vi "~ct - Type of result for 2 numeric args.vi"(6 "error in":bool, 8 "type of right":T1=enum."DBL Number", 9 "type of left":T1=enum."DBL Number") -> (0 "error out":bool, 3 "type of result":T1=enum."DBL Number", 4 "1D-2D sign":i32=-1)   [LabVIEW 2021]
doc: "::: CalcExpress Toolkit :::\nCopyright (c) 2000-2026 Konstantin Shifershteyn. All rights reserved."
uses:
  cetypes.llb/CalcExpress Data Type.ctl
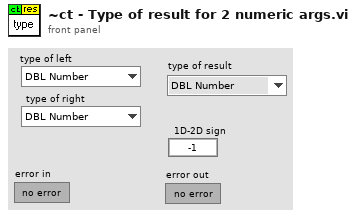
[diagram p1: front panel]
types:
  T1 = typedef "CalcExpress Data Type.ctl" = enum32{"String", "DBL Number", "identifier", "1D Array of DBL", "2D Array of DBL", "CDB Number", "1D Array of CDB", "2D Array of CDB", "1D Array of String", "2D Array of String", "Unknown data type"}
  T2 = enum8{"String", "DBL Number", "identifier", "1D Array of DBL", "2D Array of DBL", "CDB Number", "1D Array of CDB", "2D Array of CDB", "1D Array of String", "2D Array of String", "Unknown data type"}
  T3 = enum32{"String", "DBL Number", "identifier", "1D Array of DBL", "2D Array of DBL", "CDB Number", "1D Array of CDB", "2D Array of CDB", "1D Array of String", "2D Array of String", "Unknown data type"}[][]
  T4 = enum32{"String", "DBL Number", "identifier", "1D Array of DBL", "2D Array of DBL", "CDB Number", "1D Array of CDB", "2D Array of CDB", "1D Array of String", "2D Array of String", "Unknown data type"}
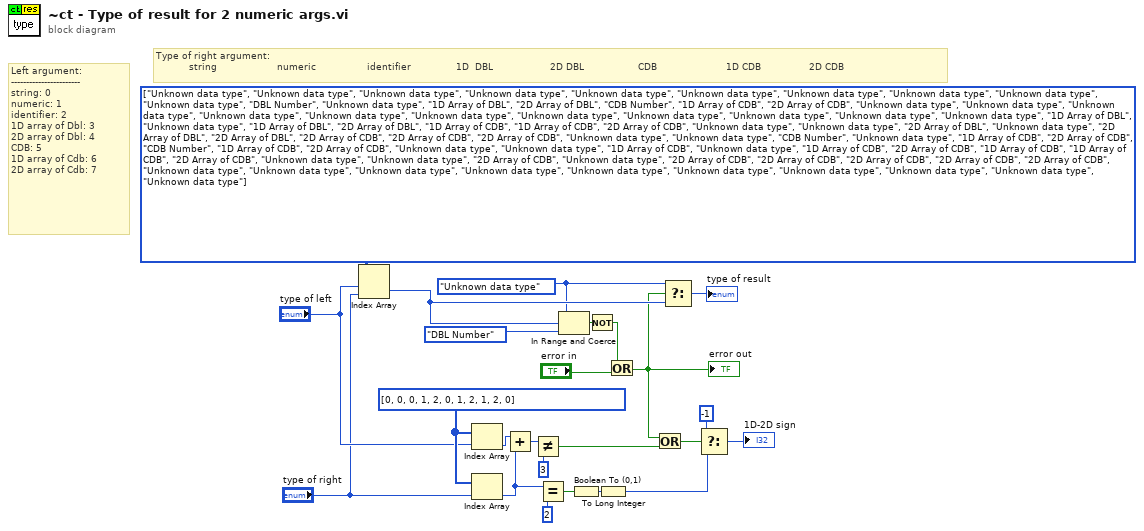
[diagram p0: block diagram]
diagram:
  w7 = i32[] [0, 0, 0, 1, 2, 0, 1, 2, 1, 2, 0]
  w18 = T2."Unknown data type" ("type of result")
  w24 = T3 [[enum."Unknown data type", enum."Unknown data type", enum."Unknown data type", enum."Unknown data type", enum."Unknown data type", enum."Unknown data type", enum."Unknown data type", enum."Unknown data type", enum."Unknown data type"], [enum."Unknown data type", enum."DBL Number", enum."Unknown data type", enum."1D Array of DBL", enum."2D Array of DBL", enum."CDB Number", enum."1D Array of CDB", enum."2D Array of CDB", enum."Unknown data type"], [enum."Unknown data type", enum."Unknown data type", enum."Unknown data type", enum."Unknown data type", enum."Unknown data type", enum."Unknown data type", enum."Unknown data type", enum."Unknown data type", enum."Unknown data type"], [enum."Unknown data type", enum."1D Array of DBL", enum."Unknown data type", enum."1D Array of DBL", enum."2D Array of DBL", enum."1D Array of CDB", enum."1D Array of CDB", enum."2D Array of CDB", enum."Unknown data type"], [enum."Unknown data type", enum."2D Array of DBL", enum."Unknown data type", enum."2D Array of DBL", enum."2D Array of DBL", enum."2D Array of CDB", enum."2D Array of CDB", enum."2D Array of CDB", enum."Unknown data type"], [enum."Unknown data type", enum."CDB Number", enum."Unknown data type", enum."1D Array of CDB", enum."2D Array of CDB", enum."CDB Number", enum."1D Array of CDB", enum."2D Array of CDB", enum."Unknown data type"], [enum."Unknown data type", enum."1D Array of CDB", enum."Unknown data type", enum."1D Array of CDB", enum."2D Array of CDB", enum."1D Array of CDB", enum."1D Array of CDB", enum."2D Array of CDB", enum."Unknown data type"], [enum."Unknown data type", enum."2D Array of CDB", enum."Unknown data type", enum."2D Array of CDB", enum."2D Array of CDB", enum."2D Array of CDB", enum."2D Array of CDB", enum."2D Array of CDB", enum."Unknown data type"], [enum."Unknown data type", enum."Unknown data type", enum."Unknown data type", enum."Unknown data type", enum."Unknown data type", enum."Unknown data type", enum."Unknown data type", enum."Unknown data type", enum."Unknown data type"]] items=["String", "DBL Number", "identifier", "1D Array of DBL", "2D Array of DBL", "CDB Number", "1D Array of CDB", "2D Array of CDB", "1D Array of String", "2D Array of String", "Unknown data type"]
  # "Type of right argument:\n           string                    numeric                 identifier               1D  DBL                   2D DBL                  CDB                       1D CDB                2D CDB"
  # "Left argument:\n-----------------------\nstring: 0\nnumeric: 1\nidentifier: 2\n1D array of Dbl: 3\n2D array of Dbl: 4\nCDB: 5\n1D array of Cdb: 6\n2D array of Cdb: 7"
  n1 = Index Array(array=w24, index (row)="type of left", index (col)="type of right") -> (element=w19:T4)
  n2 = Index Array(array=w7, index="type of left") -> (element=w8:i32)
  n3 = Index Array(array=w7, index="type of right") -> (element=w11:i32)
  n4 = Add(x=w8, y=w11) -> (x+y=w9:i32)
  n5 = Not Equal?(x=w9, y=3) -> (x != y?=w3:bool)
  n6 = Equal?(x=w11, y=2) -> (x = y?=w13:bool)
  n7 = In Range and Coerce(upper limit=w18, x=w19, lower limit=T2."DBL Number" ("type of result")) -> (In Range?=w23:bool)  [unwired: 1 out]
  n8 = Boolean To (0,1)(Boolean=w13) -> (0, 1=w14:i16)
  n9 = Not(x=w23) -> (.not. x?=w22:bool)
  n10 = To Long Integer(number=w14) -> (32bit integer=w15:i32)
  n11 = Or(x=w22, y="error in") -> (x .or. y?=w2:bool)
  "error out" <- w2
  n12 = Or(x=w2, y=w3) -> (x .or. y?=w1:bool)
  n13 = Select(t=w18, s=w2, f=w19) -> (s? t:f=→"type of result":T4)
  n14 = Select(t=-1, s=w1, f=w15) -> (s? t:f=→"1D-2D sign":i32)
